vi "Send TurnTable Processing Event.vi"(8 "error in (no error)":errorcluster caption="에러 입력(에러 없음)", 9 "숫자형":dbl, 10 "id":string, 11 "Instrument Manager 입력":refnum<class "Instrument Manager.lvclass">) -> (0 "error out":errorcluster caption="에러 출력", 3 "Instrument Manager 출력":refnum<class "Instrument Manager.lvclass">)   [LabVIEW 2023, in "Instrument Manager.lvclass"]
uses:
  Instrument Manager.lvclass
  TurnTable Processing Event.ctl
  Instrument Manager.lvclass/Instrument Manager.ctl
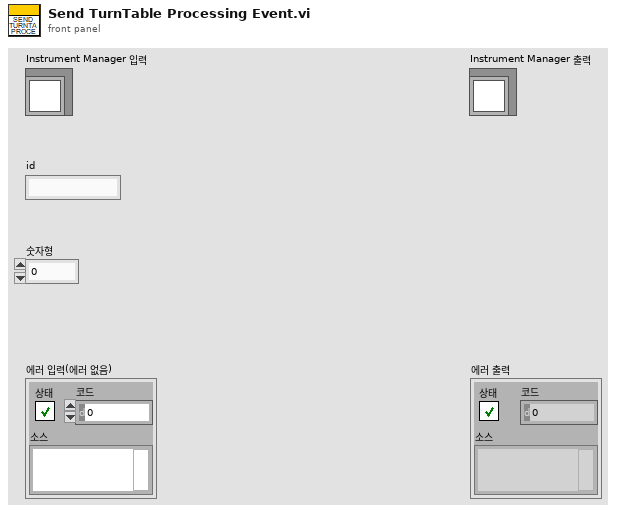
[diagram p1: front panel]
types:
  T1 = typedef "Instrument Manager.lvclass/TurnTable Processing Event.ctl" = cluster{"type":string, "id":string, "target":string, "command":string, "Params":cluster{"Current Angle":dbl}}
  T2 = cluster{"Reader Q":refnum<queue>, "Writer Q":refnum<queue>}
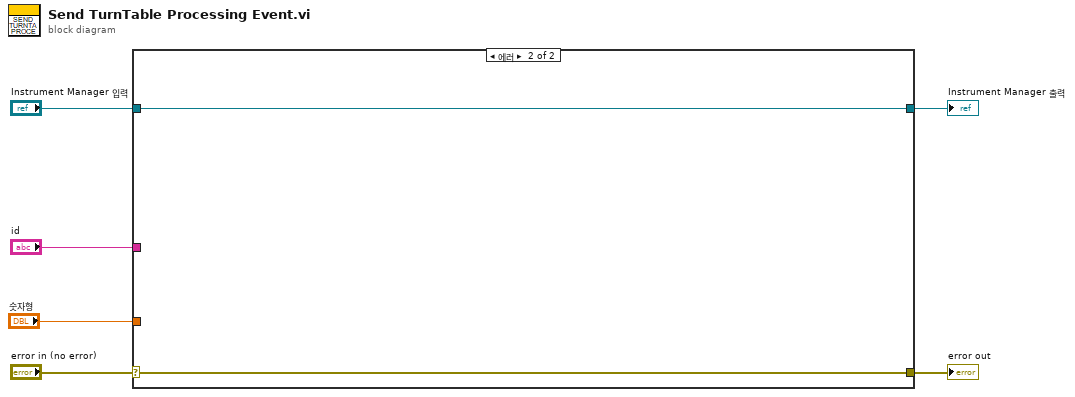
[diagram p0: block diagram]
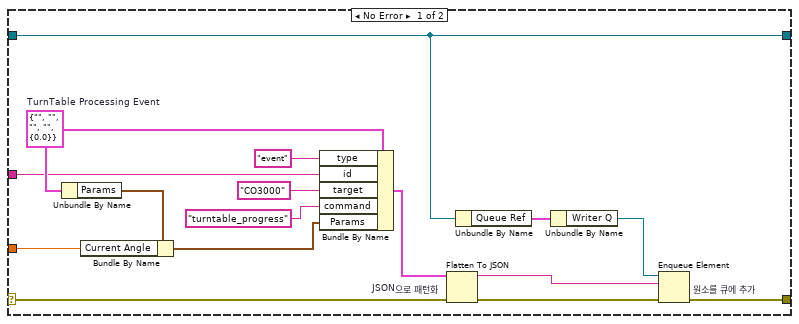
[diagram p2: hidden frame]
diagram:
  n1 = case shown="에러" "error in (no error)" {
    selector: "error in (no error)" -> [w11 w23]
    tunnel: [w9 w23] -> w5
    tunnel: [w8 w24] -> w3
    tunnel: "Instrument Manager 입력" -> [w8 w24]
    tunnel: "id" -> [w18 _]
    tunnel: "숫자형" -> [w20 _]
    frame No Error {
      w22 = T1 {"type"="", "id"="", "target"="", "command"="", "Params"={"Current Angle"=0.0}}  # TurnTable Processing Event
      n2 = Unbundle By Name(w22) -> ("Params"=w21:cluster{"Current Angle":dbl})
      n3 = Bundle By Name(cluster=w21, "Current Angle"=w20) -> (w19:cluster{"Current Angle":dbl})
      n4 = Bundle By Name(cluster=w22, "type"="event", "id"=w18, "target"="CO3000", "command"="turntable_progress", "Params"=w19) -> (w7:T1)
      n5 = Flatten To JSON "JSON으로 패턴화"(anything=w7, error in (no error)=w11) -> (JSON string=w12:string, 11:w10:errorcluster)  [unwired: 1 in]
      n6 = Unbundle By Name(w8) -> ("Queue Ref"=w14:T2)
      n7 = Unbundle By Name(w14) -> ("Writer Q"=w13:refnum<queue>)
      n8 = Enqueue Element "원소를 큐에 추가"(queue=w13, element=w12, error in (no error)=w10) -> (error out=w9:errorcluster)  [unwired: 1 in, 2 out]
    }
    frame Error {
    }
  }
  "error out" <- w5
  "Instrument Manager 출력" <- w3
